vi "launch target selector.vi"(8 "error in (no error)":errorcluster, 10 "Options":string[](array[string])) -> (0 "error out":errorcluster, 1 "Canceled?":bool, 3 "Target Index":i32)   [LabVIEW 2013, in "Standard Editor.lvlib"]
uses:
  Standard Editor.lvlib
panel:
  in  "Cancel":bool
  in  "OK":bool
  in  "Select Target":i32(ring)
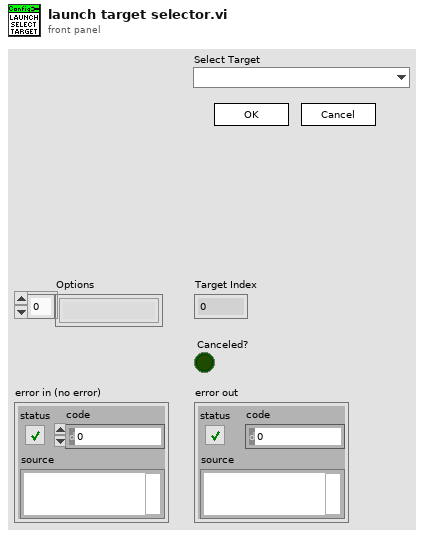
[diagram p1: front panel]
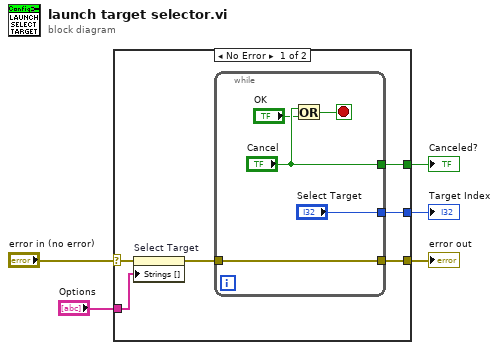
[diagram p0: block diagram]
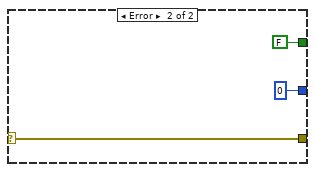
[diagram p2: hidden frame]
diagram:
  n1 = case shown="No Error" "error in (no error)" {
    selector: "error in (no error)" -> [w10 w17]
    tunnel: "Options" -> [w11 _]
    tunnel: [w8 0 ("Select Target")] -> w3
    tunnel: [w7 FALSE ("Cancel")] -> w2
    tunnel: [w6 w17] -> w1
    frame No Error {
      n2 = property on="Select Target" class="Ring (strict)"(error in=w10, "Strings []"=w11) -> (error out=w9:errorcluster)  [unwired: 1 in, 1 out]
      n3 = while {
        tunnel: w9 -> [w12]
        tunnel: ["Select Target"] -> w8
        tunnel: ["Cancel"] -> w7
        tunnel: [w12] -> w6
        stop <- w13 stop-if-true
        n4 = Or(x="Cancel", y="OK") -> (x .or. y?=w13:bool)
      }
    }
    frame Error {
    }
  }
  "Canceled?" <- w2
  "error out" <- w1
  "Target Index" <- w3
